vi "convert round OBW Measurement to TYPE Cluster Format.vi"(8 "error in (no error)":errorcluster, 10 "OBW Measurement Rounded Result":dbl[](array[numeric]), 11 "Keysight 9020A in":refnum<class "Keysight 9020A.lvclass">) -> (0 "error out":errorcluster, 2 "OBW Measurement":T1, 3 "Keysight 9020A out":refnum<class "Keysight 9020A.lvclass">)   [LabVIEW 2023, in "Spectrum Analyzer.lvlib" / "Keysight 9020A.lvclass"]
uses:
  Keysight 9020A.lvclass
  Keysight 9020A.lvclass/Keysight 9020A.ctl
  TYPE DEFINITION/SA Measurement Class/TYPE OBW Measurement.ctl
  Spectrum Analyzer.lvlib
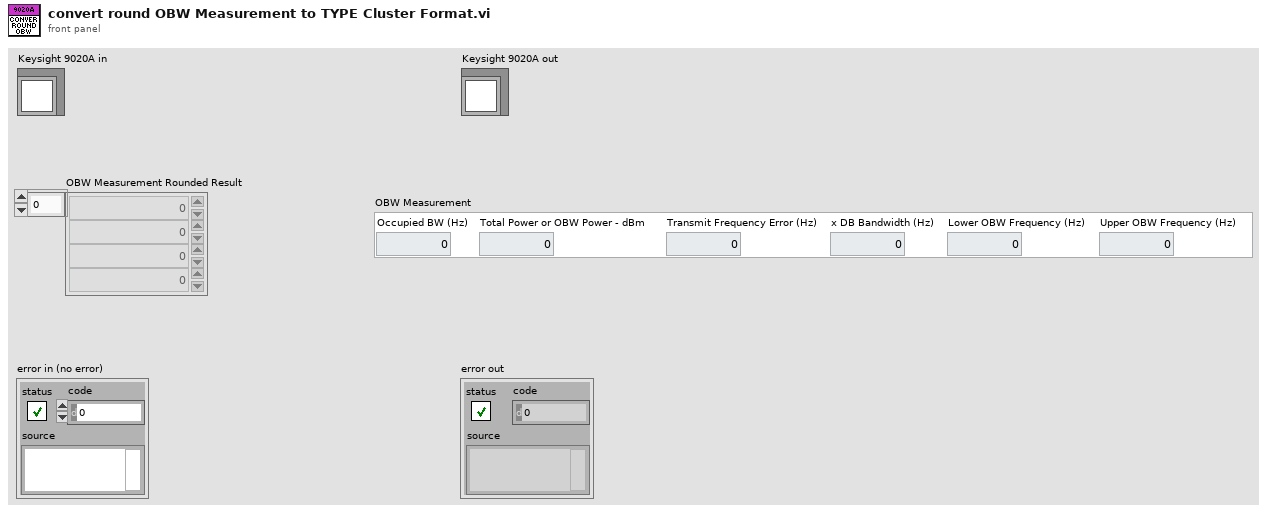
[diagram p1: front panel]
types:
  T1 = typedef "Spectrum Analyzer.lvlib/TYPE OBW Measurement.ctl" = cluster{"Occupied BW (Hz)":dbl, "Total Power or OBW Power - dBm":dbl, "Transmit Frequency Error (Hz)":dbl, "x DB Bandwidth (Hz)":dbl, "Lower OBW Frequency (Hz)":dbl, "Upper OBW Frequency (Hz)":dbl}
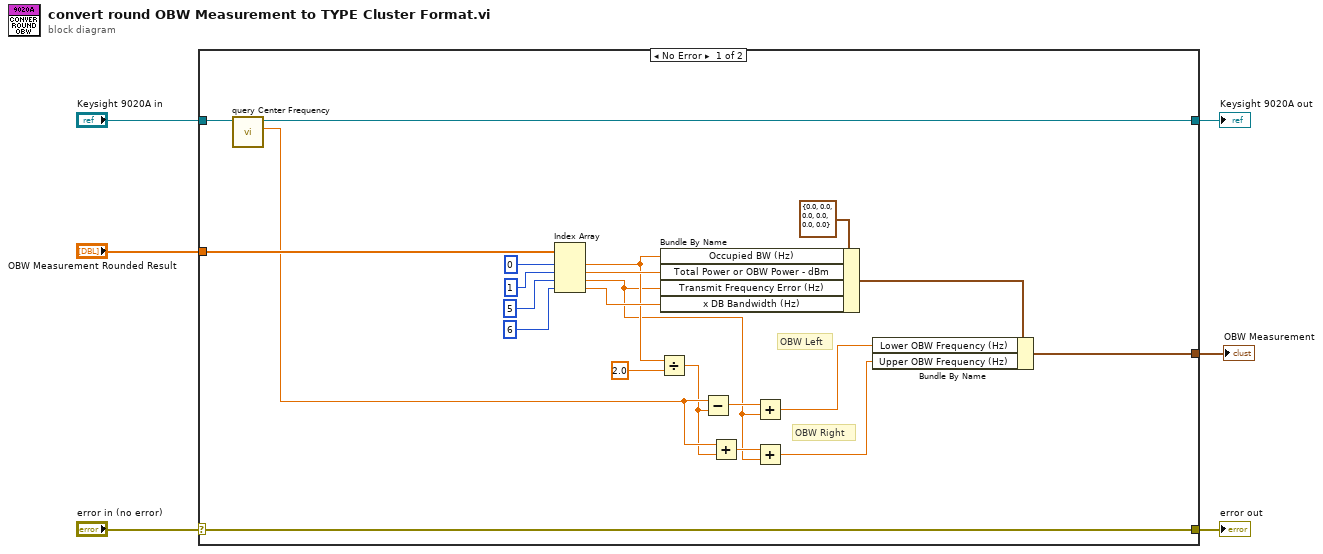
[diagram p0: block diagram]
diagram:
  n1 = case shown="No Error" "error in (no error)" {
    selector: "error in (no error)" -> [w28 w30]
    tunnel: [w28 w30] -> w5
    tunnel: [w25 w29] -> w3
    tunnel: "Keysight 9020A in" -> [w26 w29]
    tunnel: "OBW Measurement Rounded Result" -> [w27 _]
    tunnel: [w7 _] -> w1
    frame No Error {
      # "OBW Right"
      # "OBW Left"
      n2 = call-dynamic "query Center Frequency.vi"("Keysight 9020A in"=w26) -> ("Center Frequency (Hz)"=w24:dbl, "Keysight 9020A out"=w25:refnum<class "Keysight 9020A.lvclass">)  [unwired: 8 in, 1 out]
      n3 = Index Array(array=w27, index #1=0 ("index"), index #2=1 ("index"), index #3=5 ("index"), index #4=6 ("index")) -> (element #1=w16:dbl, element #2=w20:dbl, element #3=w11:dbl, element #4=w17:dbl)
      n4 = Divide(x=w16, y=2.0) -> (x/y=w12:dbl)
      n5 = Bundle By Name(cluster=T1 {"Occupied BW (Hz)"=0.0, "Total Power or OBW Power - dBm"=0.0, "Transmit Frequency Error (Hz)"=0.0, "x DB Bandwidth (Hz)"=0.0, "Lower OBW Frequency (Hz)"=0.0, "Upper OBW Frequency (Hz)"=0.0} ("OBW Measurement 2"), "Occupied BW (Hz)"=w16, "Total Power or OBW Power - dBm"=w20, "Transmit Frequency Error (Hz)"=w11, "x DB Bandwidth (Hz)"=w17) -> (w10:T1)
      n6 = Subtract(x=w24, y=w12) -> (x-y=w14:dbl)
      n7 = Add(x=w24, y=w12) -> (x+y=w13:dbl)
      n8 = Add(x=w14, y=w11) -> (x+y=w9:dbl)
      n9 = Add(x=w13, y=w11) -> (x+y=w8:dbl)
      n10 = Bundle By Name(cluster=w10, "Lower OBW Frequency (Hz)"=w9, "Upper OBW Frequency (Hz)"=w8) -> (w7:T1)
    }
    frame Error {
    }
  }
  "error out" <- w5
  "Keysight 9020A out" <- w3
  "OBW Measurement" <- w1
